vi "Find Parse State Queue from While Loop.vi"(8 "error in (no error)":errorcluster, 11 "WhileLoop in":refnum<vi>) -> (0 "error out":errorcluster, 1 "CaseStructure":refnum<vi>, 2 "Parse State Queue":refnum<vi>)   [LabVIEW 2020, in "JKI State Machine API.lvlib" / "JKI SM.lvclass"]
uses:
  JKI SM.lvclass
  JKI SM.lvclass/JKI SM.ctl
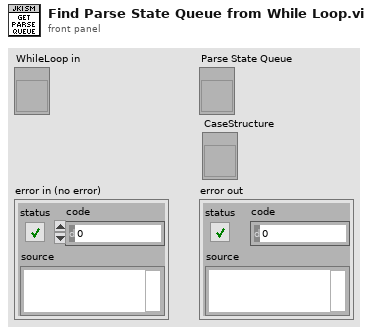
[diagram p1: front panel]
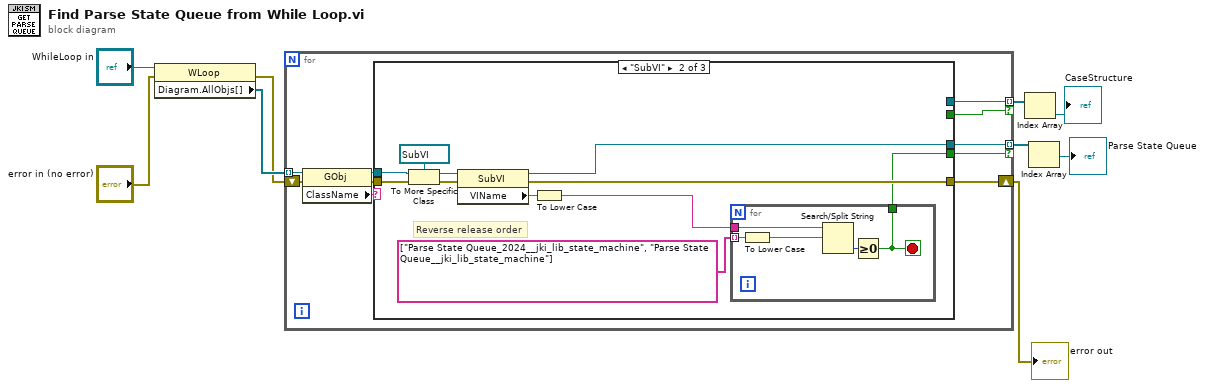
[diagram p0: block diagram]
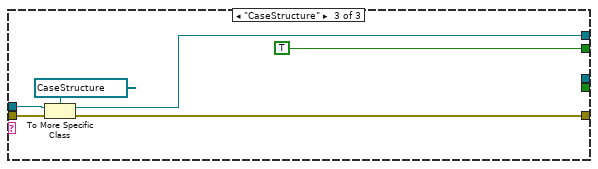
[diagram p3: hidden frame]
diagram:
  n1 = property class="WLoop"(reference="WhileLoop in", error in="error in (no error)") -> (error out=w6:errorcluster, "Diagram.AllObjs[]"=w9:refnum<vi>[])  [unwired: 1 out]
  n2 = for {
    tunnel: w9 -> [w19] mode=indexing
    shift-right: [w14] -> w5
    shift-left: w6 -> [w15]
    tunnel: [w13] -> w2 mode=indexing if=w10
    tunnel: [w12] -> w4 mode=indexing if=w11
    n3 = property class="GObj"(reference=w19, error in=w15) -> (reference out=w17:refnum<vi>, error out=w16:errorcluster, "ClassName"=w18:string)
    n4 = case shown="\"SubVI\"" w18 {
      tunnel: w17 -> [_ w30 w41]
      tunnel: w16 -> [w20 w29 w40]
      tunnel: [w20 w25 w39] -> w14
      tunnel: [_ w24 _] -> w13
      tunnel: [_ _ w38] -> w12
      tunnel: [_ _ TRUE] -> w11
      tunnel: [_ w22 _] -> w10
      frame Default {
      }
      frame "SubVI" {
        # "Reverse release order"
        n5 = To More Specific Class(target class=refnum<vi> refnum ("SubVI Refnum"), reference=w30, error in=w29) -> (specific class reference=w28:refnum<vi>, error out=w27:errorcluster)
        n6 = property class="SubVI"(reference=w28, error in=w27) -> (reference out=w24:refnum<vi>, error out=w25:errorcluster, "VIName"=w26:string)
        n7 = To Lower Case(string=w26) -> (all lower case string=w23:string)
        n8 = for {
          tunnel: w23 -> [w35]
          tunnel: [w32] -> w22
          tunnel: string[] ["Parse State Queue_2024__jki_lib_state_machine", "Parse State Queue__jki_lib_state_machine"] ("VI Name") -> [w33] mode=indexing
          stop <- w32 stop-if-true
          n9 = To Lower Case(string=w33) -> (all lower case string=w36:string)
          n10 = Search/Split String(string=w35, search string/char (-)=w36) -> (offset of match=w34:i32)  [unwired: 1 in, 2 out]
          n11 = Greater Or Equal To 0?(x=w34) -> (x >= 0?=w32:bool)
        }
      }
      frame "CaseStructure" {
        n12 = To More Specific Class(target class=refnum<vi> refnum ("CaseSel Refnum"), reference=w41, error in=w40) -> (specific class reference=w38:refnum<vi>, error out=w39:errorcluster)
      }
    }
  }
  "error out" <- w5
  n13 = Index Array(array=w4) -> (element=→"CaseStructure":refnum<vi>)  [unwired: 1 in]
  n14 = Index Array(array=w2) -> (element=→"Parse State Queue":refnum<vi>)  [unwired: 1 in]
